vi "LabVIEW.Main.Main_Program.vi"() -> ()   [LabVIEW 2019]
uses:
  LabVIEW.Type Definitions/LabVIEW.Main.Main_Program_Command.ctl
  LabVIEW.Type Definitions/LabVIEW.HTTPs_Client.Command.ctl
  <vilib>/JDP Science/JSONtext/JSONtext.lvlib
panel:
  out "User":T1(array[cluster])
  in  "Test User":bool
  out "Vorgang/Fertigmeldung":T1(array[cluster])
  in  "Test Vorgang/Fertigmeldung":bool
  out "Product/Serial Number":T1(array[cluster])
  in  "Test Product/Serial Number":bool
  out "Label":T1(array[cluster])
  in  "Test Label":bool
  in  "Test Authentication":bool
  out "Authentication":T1(array[cluster])
  out "Größe(n)":i32[](array[numeric])
  out "Table":string[][](table)
  in  "stop":bool caption="Stopp"
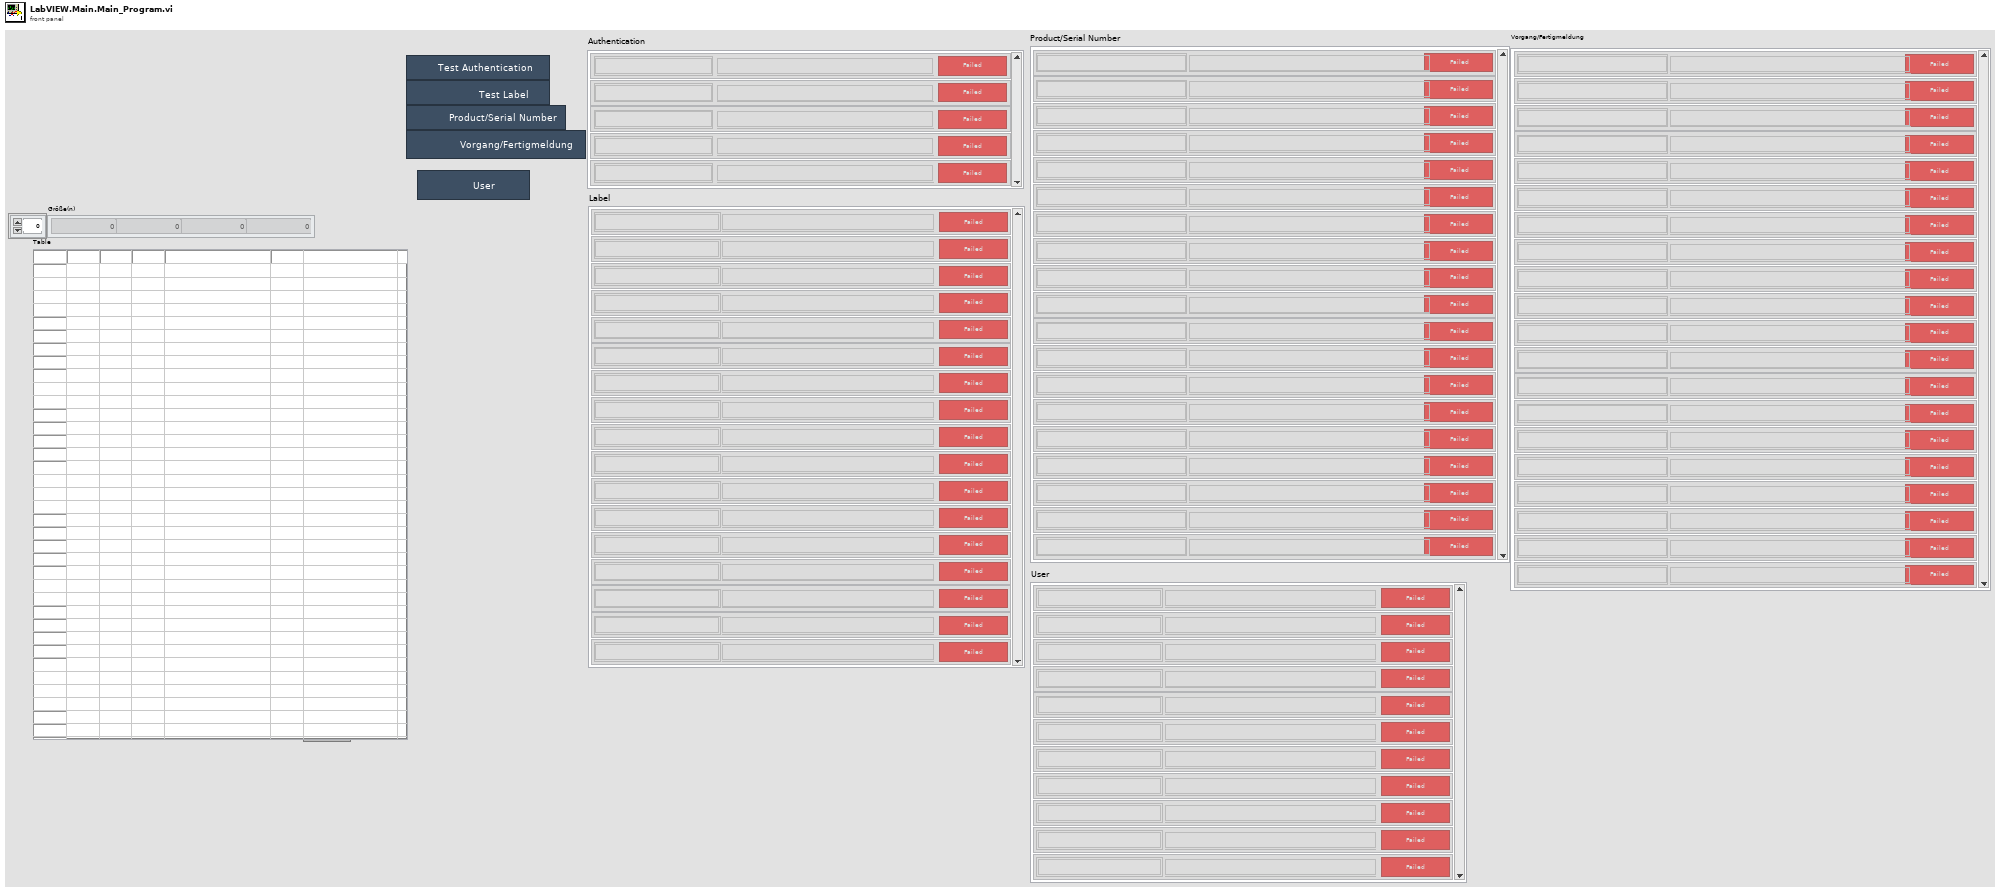
[diagram p1: front panel]
types:
  T1 = cluster{"API Name":string, "API":string, "LED":bool}[]
  T2 = typedef "LabVIEW.Main.Main_Program_Command.ctl" = enum16{"Test Authentication", "Test Label", "Test Product/Serial Number", "Test Vorgang/Fertigmeldung", "Test User"}
  T3 = typedef "LabVIEW.HTTPs_Client.Command.ctl" = enum16{"Initialize HTTPS", "Authentication: Creat a token", "Authentication: Get all tokens", "Authentication: Revoke the token", "Label: Creat a label configuration", "Label: Get all configured labels", "Label: Update the label configuration", "Label: Delete the label configuration", "Label: Creat a colour ribbon", "Label: Update the colour ribbon", "Label: Get all colour ribbons", "Label: Delete the colour ribbon", "Label: Creat a label tape", "Label: Update the label tape", "Label: Get all label tapes", "Label: Delete the label tape", "Label: Get all label parameters", "Product: Get all product informations", "Product: Get all reading steps", "Seriennummer: Update the info text", "Seriennummer: Set all step states open", "Seriennummer: Update step states", "Seriennummer: Get data and steps", "Seriennummer: Get all label configurations", "Seriennummer: Create a text report(Prüfbericht)", "Seriennummer: Get the text report(Prüfbericht)", "Seriennummer: Delete the text report(Prüfbericht)", "Seriennummer: Upload a document(txt file)", "Seriennummer: Get the document", "Seriennummer: Get the document thumbnail", "Seriennummer: Delete the document", "Seriennummer: Bulk lookup", "Vorgang: Update the description text", "Vorgang: Migrate serial numbers to a Vorgang", "Vorgang: Migrate serial numbers to a product revision", "Vorgang: Update step states", "Vorgang: Create test reports(Prüfprotokoll)", "Vorgang: Get basic data", "Vorgang: Get serial number data and steps", "Vorgang: Get all serial numbers", "Vorgang: Generate a CSV file", "Vorgang: Generate an XLSX file", "Vorgang: Get a CSV file(Fertigmeldung report)", "Fertigmeldung: Create a Fertigmeldung", "Fertigmeldung: Revert the Fertigmeldung", "User: Get all users", "User: Update an user", "User: Get a single user", "User: Get all user roles", "User: Update a user role", "User: Get a single user role", "User: Get all permissions", "Search: Get Vorgang/Produkt combinations", "Search: Get Vorgang/Produkt/SN combinations", "Search: Get Seriennummern by Vorgang and Produkt", "Search: Lookup Vorgang", "MAC addresses: Get all reserved MAC addresses", "MAC addresses: Get the most recently reserved MAC addresses", "MAC addresses: Get data for a MAC address", "MAC addresses: Reserve MAC addresses for a Seriennummer", "MAC addresses: Mark a reserved MAC address as flashed", "Deinitialize HTTPs"}
  T4 = enum16{"read csv", "clear csv", "read xlsx", "clear xlsx"}
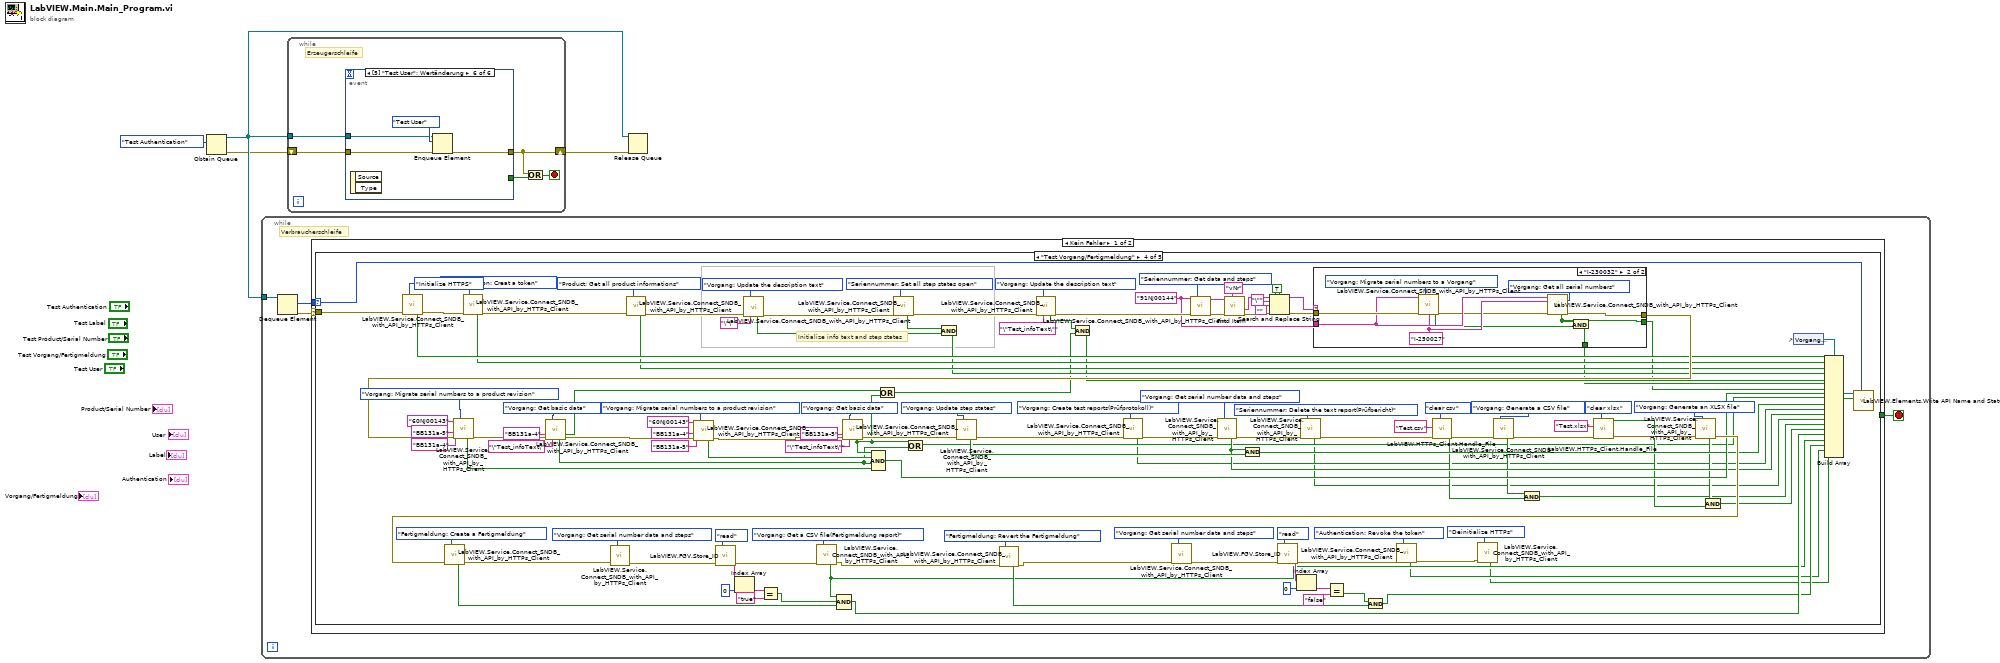
[diagram p0: block diagram]
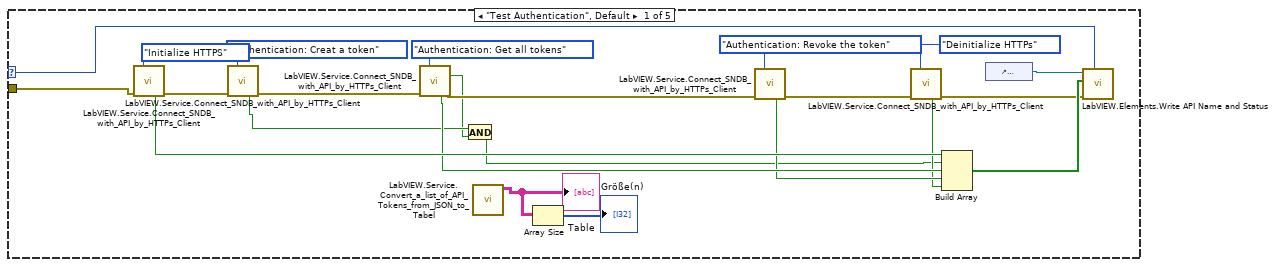
[diagram p2: hidden frame]
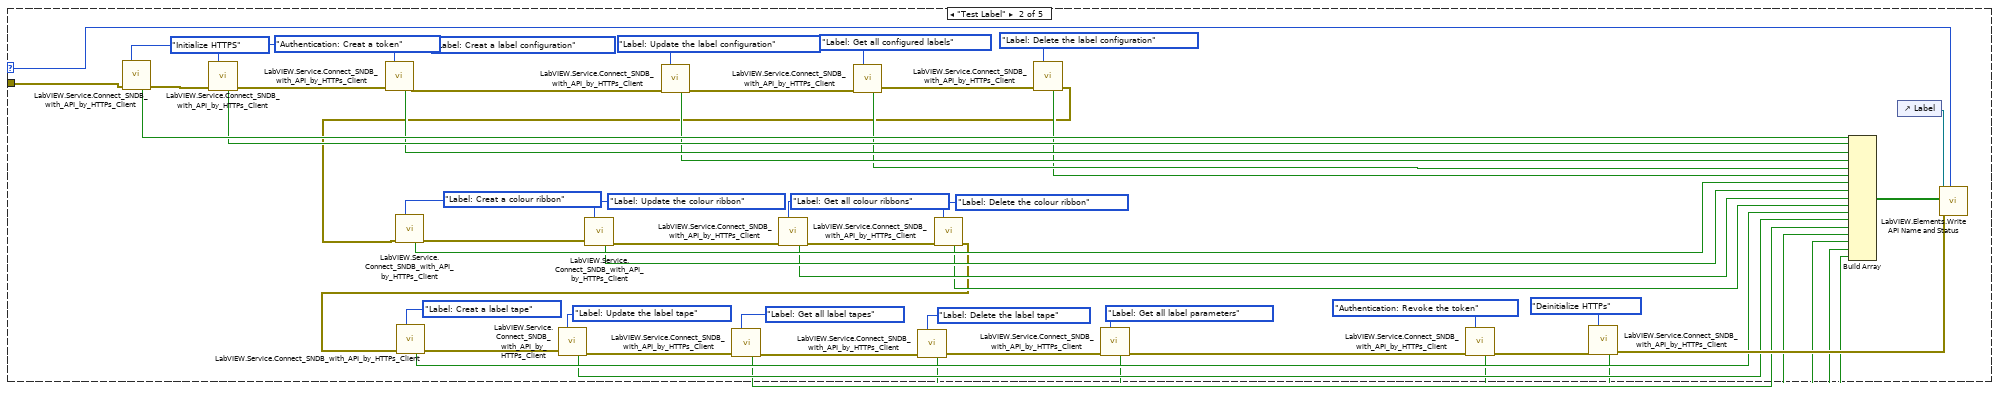
[diagram p3: hidden frame]
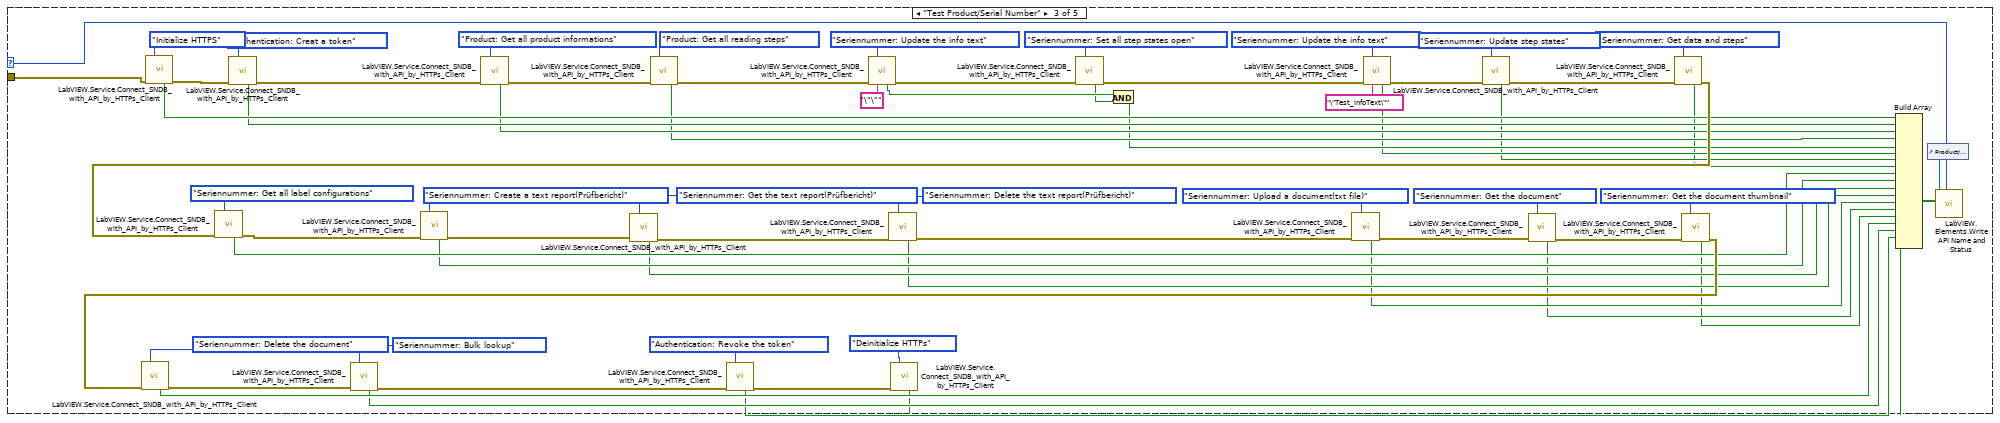
[diagram p4: hidden frame]
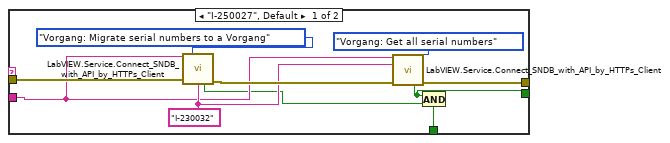
[diagram p5: hidden frame]
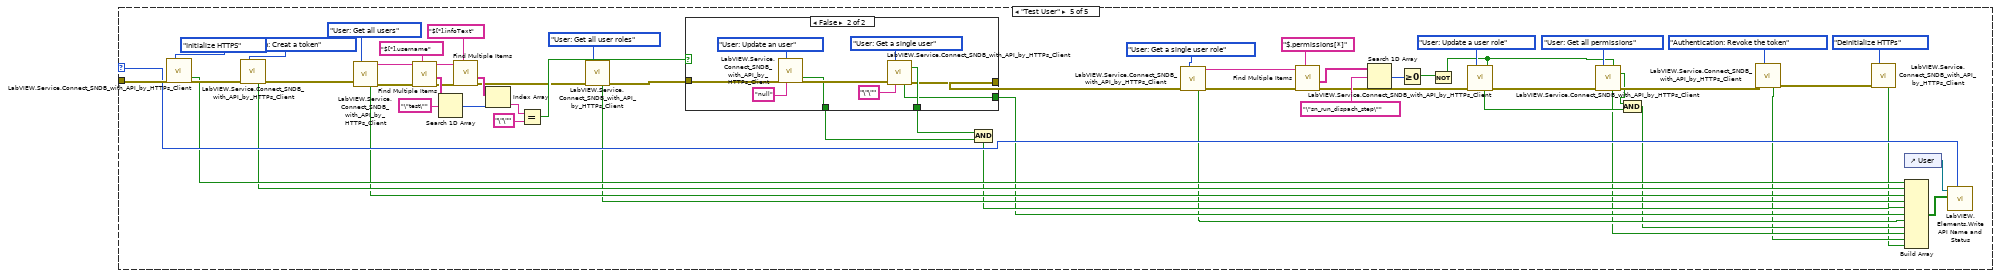
[diagram p6: hidden frame]
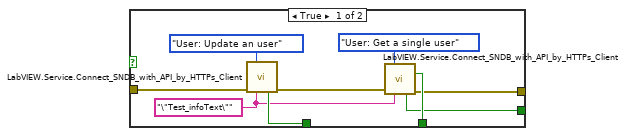
[diagram p7: hidden frame]
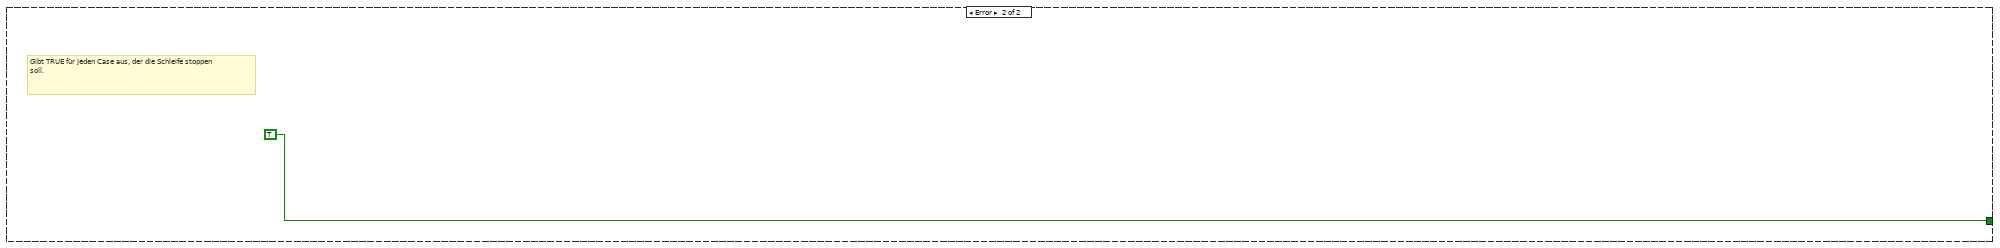
[diagram p8: hidden frame]
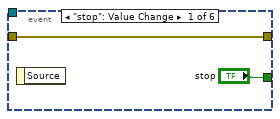
[diagram p9: hidden frame]
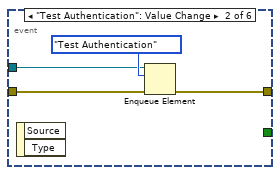
[diagram p10: hidden frame]
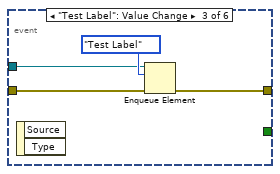
[diagram p11: hidden frame]
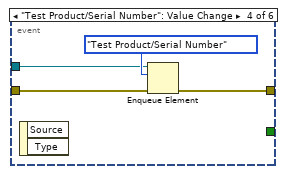
[diagram p12: hidden frame]
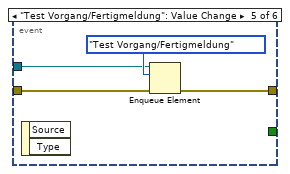
[diagram p13: hidden frame]
diagram:
  n1 = Obtain Queue(element data type=LabVIEW.Main.Main_Program_Command."Test Authentication" ("Command")) -> (queue out=w2:refnum<queue>, error out=w1:errorcluster)  [unwired: 4 in, 1 out]
  n2 = while {
    tunnel: w2 -> [w8]
    stop <- w5 stop-if-true
    # "Verbraucherschleife"
    n3 = Dequeue Element(queue=w8) -> (element=w6:T2, error out=w7:errorcluster)  [unwired: 2 in, 2 out]
    n4 = case shown="Kein Fehler" w7 {
      selector: w7 -> [w9 _]
      tunnel: w6 -> [w10 _]
      tunnel: [_ TRUE] -> w5
      frame No Error {
        n5 = case shown="\"Test Vorgang/Fertigmeldung\"" w10 {
          selector: w10 -> [w14 w34 w112 w199 w333]
          tunnel: w9 -> [w33 w88 w151 w280 w357]
          frame "Test Authentication", Default {
            n6 = call "LabVIEW.Service.Connect_SNDB_with_API_by_HTTPs_Client.vi"("Command"=LabVIEW.HTTPs_Client.Command."Initialize HTTPS", "error in (no error)"=w33) -> ("Successful?"=w26:bool, "error out"=w32:errorcluster)  [unwired: 7 in, 5 out]
            n7 = call "LabVIEW.Service.Connect_SNDB_with_API_by_HTTPs_Client.vi"("Command"=LabVIEW.HTTPs_Client.Command."Authentication: Creat a token", "error in (no error)"=w32) -> ("Successful?"=w13:bool, "error out"=w29:errorcluster)  [unwired: 7 in, 5 out]
            n8 = call "LabVIEW.Service.Connect_SNDB_with_API_by_HTTPs_Client.vi"("Command"=LabVIEW.HTTPs_Client.Command."Authentication: Get all tokens", "error in (no error)"=w29) -> ("Test other steps"=w12:bool, "Successful?"=w25:bool, "error out"=w28:errorcluster)  [unwired: 7 in, 4 out]
            n9 = And(x=w13, y=w12) -> (x .and. y?=w11:bool)
            n10 = call "LabVIEW.Service.Convert_a_list_of_API_Tokens_from_JSON_to_Tabel.vi"() -> ("API Tokens"=w31:string[][])  [unwired: 10 in, 1 out]
            "Table" <- w31
            n11 = Array Size(array=w31) -> (size(s)=→"Größe(n)":i32[])
            n12 = call "LabVIEW.Service.Connect_SNDB_with_API_by_HTTPs_Client.vi"("Command"=LabVIEW.HTTPs_Client.Command."Authentication: Revoke the token", "error in (no error)"=w28) -> ("Successful?"=w24:bool, "error out"=w22:errorcluster)  [unwired: 7 in, 5 out]
            n13 = call "LabVIEW.Service.Connect_SNDB_with_API_by_HTTPs_Client.vi"("Command"=LabVIEW.HTTPs_Client.Command."Deinitialize HTTPs", "error in (no error)"=w22) -> ("Successful?"=w21:bool, "error out"=w20:errorcluster)  [unwired: 7 in, 5 out]
            n14 = Build Array(w26, w11, w25, w24, w21) -> (w23:bool[])
            n15 = control-ref of="Authentication"() -> (w27:refnum<vi>)
            n16 = call "LabVIEW.Elements.Write API Name and Status.vi"("Command"=w14, "Fehler (Eingang, kein Fehler)"=w20, "Status[]"=w23, "Array Reference"=w27) -> ()  [unwired: 7 in, 1 out]
          }
          frame "Test Label" {
            n17 = call "LabVIEW.Service.Connect_SNDB_with_API_by_HTTPs_Client.vi"("Command"=LabVIEW.HTTPs_Client.Command."Initialize HTTPS", "error in (no error)"=w88) -> ("Successful?"=w84:bool, "error out"=w87:errorcluster)  [unwired: 7 in, 5 out]
            n18 = call "LabVIEW.Service.Connect_SNDB_with_API_by_HTTPs_Client.vi"("Command"=LabVIEW.HTTPs_Client.Command."Authentication: Creat a token", "error in (no error)"=w87) -> ("Successful?"=w83:bool, "error out"=w86:errorcluster)  [unwired: 7 in, 5 out]
            n19 = call "LabVIEW.Service.Connect_SNDB_with_API_by_HTTPs_Client.vi"("Command"=LabVIEW.HTTPs_Client.Command."Label: Creat a label configuration", "error in (no error)"=w86) -> ("Successful?"=w82:bool, "error out"=w85:errorcluster)  [unwired: 7 in, 5 out]
            n20 = call "LabVIEW.Service.Connect_SNDB_with_API_by_HTTPs_Client.vi"("Command"=LabVIEW.HTTPs_Client.Command."Label: Update the label configuration", "error in (no error)"=w85) -> ("Successful?"=w81:bool, "error out"=w79:errorcluster)  [unwired: 7 in, 5 out]
            n21 = call "LabVIEW.Service.Connect_SNDB_with_API_by_HTTPs_Client.vi"("Command"=LabVIEW.HTTPs_Client.Command."Label: Get all configured labels", "error in (no error)"=w79) -> ("Successful?"=w78:bool, "error out"=w73:errorcluster)  [unwired: 7 in, 5 out]
            n22 = call "LabVIEW.Service.Connect_SNDB_with_API_by_HTTPs_Client.vi"("Command"=LabVIEW.HTTPs_Client.Command."Label: Delete the label configuration", "error in (no error)"=w73) -> ("Successful?"=w67:bool, "error out"=w60:errorcluster)  [unwired: 7 in, 5 out]
            n23 = call "LabVIEW.Service.Connect_SNDB_with_API_by_HTTPs_Client.vi"("Command"=LabVIEW.HTTPs_Client.Command."Label: Creat a colour ribbon", "error in (no error)"=w60) -> ("Successful?"=w56:bool, "error out"=w59:errorcluster)  [unwired: 7 in, 5 out]
            n24 = call "LabVIEW.Service.Connect_SNDB_with_API_by_HTTPs_Client.vi"("Command"=LabVIEW.HTTPs_Client.Command."Label: Update the colour ribbon", "error in (no error)"=w59) -> ("Successful?"=w55:bool, "error out"=w58:errorcluster)  [unwired: 7 in, 5 out]
            n25 = call "LabVIEW.Service.Connect_SNDB_with_API_by_HTTPs_Client.vi"("Command"=LabVIEW.HTTPs_Client.Command."Label: Get all colour ribbons", "error in (no error)"=w58) -> ("Successful?"=w54:bool, "error out"=w57:errorcluster)  [unwired: 7 in, 5 out]
            n26 = call "LabVIEW.Service.Connect_SNDB_with_API_by_HTTPs_Client.vi"("Command"=LabVIEW.HTTPs_Client.Command."Label: Delete the colour ribbon", "error in (no error)"=w57) -> ("Successful?"=w53:bool, "error out"=w45:errorcluster)  [unwired: 7 in, 5 out]
            n27 = call "LabVIEW.Service.Connect_SNDB_with_API_by_HTTPs_Client.vi"("Command"=LabVIEW.HTTPs_Client.Command."Label: Creat a label tape", "error in (no error)"=w45) -> ("Successful?"=w44:bool, "error out"=w48:errorcluster)  [unwired: 7 in, 5 out]
            n28 = call "LabVIEW.Service.Connect_SNDB_with_API_by_HTTPs_Client.vi"("Command"=LabVIEW.HTTPs_Client.Command."Label: Update the label tape", "error in (no error)"=w48) -> ("Successful?"=w43:bool, "error out"=w47:errorcluster)  [unwired: 7 in, 5 out]
            n29 = call "LabVIEW.Service.Connect_SNDB_with_API_by_HTTPs_Client.vi"("Command"=LabVIEW.HTTPs_Client.Command."Label: Get all label tapes", "error in (no error)"=w47) -> ("Successful?"=w42:bool, "error out"=w46:errorcluster)  [unwired: 7 in, 5 out]
            n30 = call "LabVIEW.Service.Connect_SNDB_with_API_by_HTTPs_Client.vi"("Command"=LabVIEW.HTTPs_Client.Command."Label: Delete the label tape", "error in (no error)"=w46) -> ("Successful?"=w41:bool, "error out"=w40:errorcluster)  [unwired: 7 in, 5 out]
            n31 = call "LabVIEW.Service.Connect_SNDB_with_API_by_HTTPs_Client.vi"("Command"=LabVIEW.HTTPs_Client.Command."Label: Get all label parameters", "error in (no error)"=w40) -> ("Successful?"=w37:bool, "error out"=w39:errorcluster)  [unwired: 7 in, 5 out]
            n32 = call "LabVIEW.Service.Connect_SNDB_with_API_by_HTTPs_Client.vi"("Command"=LabVIEW.HTTPs_Client.Command."Authentication: Revoke the token", "error in (no error)"=w39) -> ("Successful?"=w36:bool, "error out"=w70:errorcluster)  [unwired: 7 in, 5 out]
            n33 = call "LabVIEW.Service.Connect_SNDB_with_API_by_HTTPs_Client.vi"("Command"=LabVIEW.HTTPs_Client.Command."Deinitialize HTTPs", "error in (no error)"=w70) -> ("Successful?"=w35:bool, "error out"=w68:errorcluster)  [unwired: 7 in, 5 out]
            n34 = Build Array(w84, w83, w82, w81, w78, w67, w56, w55, w54, w53, w44, w43, w42, w41, w37, w36, w35) -> (w80:bool[])
            n35 = control-ref of="Label"() -> (w69:refnum<vi>)
            n36 = call "LabVIEW.Elements.Write API Name and Status.vi"("Command"=w34, "Fehler (Eingang, kein Fehler)"=w68, "Status[]"=w80, "Array Reference"=w69) -> ()  [unwired: 7 in, 1 out]
          }
          frame "Test Product/Serial Number" {
            n37 = call "LabVIEW.Service.Connect_SNDB_with_API_by_HTTPs_Client.vi"("Command"=LabVIEW.HTTPs_Client.Command."Initialize HTTPS", "error in (no error)"=w151) -> ("Successful?"=w110:bool, "error out"=w154:errorcluster)  [unwired: 7 in, 5 out]
            n38 = call "LabVIEW.Service.Connect_SNDB_with_API_by_HTTPs_Client.vi"("Command"=LabVIEW.HTTPs_Client.Command."Authentication: Creat a token", "error in (no error)"=w154) -> ("Successful?"=w109:bool, "error out"=w148:errorcluster)  [unwired: 7 in, 5 out]
            n39 = call "LabVIEW.Service.Connect_SNDB_with_API_by_HTTPs_Client.vi"("Command"=LabVIEW.HTTPs_Client.Command."Product: Get all product informations", "error in (no error)"=w148) -> ("Successful?"=w108:bool, "error out"=w147:errorcluster)  [unwired: 7 in, 5 out]
            n40 = call "LabVIEW.Service.Connect_SNDB_with_API_by_HTTPs_Client.vi"("Command"=LabVIEW.HTTPs_Client.Command."Product: Get all reading steps", "error in (no error)"=w147) -> ("Successful?"=w107:bool, "error out"=w144:errorcluster)  [unwired: 7 in, 5 out]
            n41 = call "LabVIEW.Service.Connect_SNDB_with_API_by_HTTPs_Client.vi"("Command"=LabVIEW.HTTPs_Client.Command."Seriennummer: Update the info text", "error in (no error)"=w144, "Info text"="\"\"" ("SN: Info text")) -> ("Successful?"=w106:bool, "error out"=w142:errorcluster)  [unwired: 6 in, 5 out]
            n42 = call "LabVIEW.Service.Connect_SNDB_with_API_by_HTTPs_Client.vi"("Command"=LabVIEW.HTTPs_Client.Command."Seriennummer: Set all step states open", "error in (no error)"=w142) -> ("Successful?"=w105:bool, "error out"=w140:errorcluster)  [unwired: 7 in, 5 out]
            n43 = And(x=w106, y=w105) -> (x .and. y?=w104:bool)
            n44 = call "LabVIEW.Service.Connect_SNDB_with_API_by_HTTPs_Client.vi"("Command"=LabVIEW.HTTPs_Client.Command."Seriennummer: Update the info text", "error in (no error)"=w140, "Info text"="\"Test_infoText\"" ("SN: Info text")) -> ("Successful?"=w103:bool, "error out"=w138:errorcluster)  [unwired: 6 in, 5 out]
            n45 = call "LabVIEW.Service.Connect_SNDB_with_API_by_HTTPs_Client.vi"("Command"=LabVIEW.HTTPs_Client.Command."Seriennummer: Update step states", "error in (no error)"=w138) -> ("Successful?"=w102:bool, "error out"=w136:errorcluster)  [unwired: 7 in, 5 out]
            n46 = call "LabVIEW.Service.Connect_SNDB_with_API_by_HTTPs_Client.vi"("Command"=LabVIEW.HTTPs_Client.Command."Seriennummer: Get data and steps", "error in (no error)"=w136) -> ("Successful?"=w101:bool, "error out"=w115:errorcluster)  [unwired: 7 in, 5 out]
            n47 = call "LabVIEW.Service.Connect_SNDB_with_API_by_HTTPs_Client.vi"("Command"=LabVIEW.HTTPs_Client.Command."Seriennummer: Get all label configurations", "error in (no error)"=w115) -> ("Successful?"=w100:bool, "error out"=w132:errorcluster)  [unwired: 7 in, 5 out]
            n48 = call "LabVIEW.Service.Connect_SNDB_with_API_by_HTTPs_Client.vi"("Command"=LabVIEW.HTTPs_Client.Command."Seriennummer: Create a text report(Prüfbericht)", "error in (no error)"=w132) -> ("Successful?"=w99:bool, "error out"=w131:errorcluster)  [unwired: 7 in, 5 out]
            n49 = call "LabVIEW.Service.Connect_SNDB_with_API_by_HTTPs_Client.vi"("Command"=LabVIEW.HTTPs_Client.Command."Seriennummer: Get the text report(Prüfbericht)", "error in (no error)"=w131) -> ("Successful?"=w98:bool, "error out"=w129:errorcluster)  [unwired: 7 in, 5 out]
            n50 = call "LabVIEW.Service.Connect_SNDB_with_API_by_HTTPs_Client.vi"("Command"=LabVIEW.HTTPs_Client.Command."Seriennummer: Delete the text report(Prüfbericht)", "error in (no error)"=w129) -> ("Successful?"=w97:bool, "error out"=w128:errorcluster)  [unwired: 7 in, 5 out]
            n51 = call "LabVIEW.Service.Connect_SNDB_with_API_by_HTTPs_Client.vi"("Command"=LabVIEW.HTTPs_Client.Command."Seriennummer: Upload a document(txt file)", "error in (no error)"=w128) -> ("Successful?"=w96:bool, "error out"=w126:errorcluster)  [unwired: 7 in, 5 out]
            n52 = call "LabVIEW.Service.Connect_SNDB_with_API_by_HTTPs_Client.vi"("Command"=LabVIEW.HTTPs_Client.Command."Seriennummer: Get the document", "error in (no error)"=w126) -> ("Successful?"=w95:bool, "error out"=w123:errorcluster)  [unwired: 7 in, 5 out]
            n53 = call "LabVIEW.Service.Connect_SNDB_with_API_by_HTTPs_Client.vi"("Command"=LabVIEW.HTTPs_Client.Command."Seriennummer: Get the document thumbnail", "error in (no error)"=w123) -> ("Successful?"=w94:bool, "error out"=w114:errorcluster)  [unwired: 7 in, 5 out]
            n54 = call "LabVIEW.Service.Connect_SNDB_with_API_by_HTTPs_Client.vi"("Command"=LabVIEW.HTTPs_Client.Command."Seriennummer: Delete the document", "error in (no error)"=w114) -> ("Successful?"=w93:bool, "error out"=w118:errorcluster)  [unwired: 7 in, 5 out]
            n55 = call "LabVIEW.Service.Connect_SNDB_with_API_by_HTTPs_Client.vi"("Command"=LabVIEW.HTTPs_Client.Command."Seriennummer: Bulk lookup", "error in (no error)"=w118) -> ("Successful?"=w92:bool, "error out"=w117:errorcluster)  [unwired: 7 in, 5 out]
            n56 = call "LabVIEW.Service.Connect_SNDB_with_API_by_HTTPs_Client.vi"("Command"=LabVIEW.HTTPs_Client.Command."Authentication: Revoke the token", "error in (no error)"=w117) -> ("Successful?"=w91:bool, "error out"=w116:errorcluster)  [unwired: 7 in, 5 out]
            n57 = call "LabVIEW.Service.Connect_SNDB_with_API_by_HTTPs_Client.vi"("Command"=LabVIEW.HTTPs_Client.Command."Deinitialize HTTPs", "error in (no error)"=w116) -> ("Successful?"=w90:bool)  [unwired: 7 in, 6 out]
            n58 = Build Array(w110, w109, w108, w107, w104, w103, w102, w101, w100, w99, w98, w97, w96, w95, w94, w93, w92, w91, w90) -> (w113:bool[])
            n59 = control-ref of="Product/Serial Number"() -> (w111:refnum<vi>)
            n60 = call "LabVIEW.Elements.Write API Name and Status.vi"("Command"=w112, "Status[]"=w113, "Array Reference"=w111) -> ()  [unwired: 8 in, 1 out]
          }
          frame "Test Vorgang/Fertigmeldung" {
            w267 = TRUE ("Alle ersetzen? (F)")
            w261 = "91NJ00144" ("SN")
            # "Initialize info text and step states"
            n61 = call "LabVIEW.Service.Connect_SNDB_with_API_by_HTTPs_Client.vi"("Command"=LabVIEW.HTTPs_Client.Command."Initialize HTTPS", "error in (no error)"=w280) -> ("Successful?"=w197:bool, "error out"=w283:errorcluster)  [unwired: 7 in, 5 out]
            n62 = call "LabVIEW.Service.Connect_SNDB_with_API_by_HTTPs_Client.vi"("Command"=LabVIEW.HTTPs_Client.Command."Authentication: Creat a token", "error in (no error)"=w283) -> ("Successful?"=w196:bool, "error out"=w249:errorcluster)  [unwired: 7 in, 5 out]
            n63 = call "LabVIEW.Service.Connect_SNDB_with_API_by_HTTPs_Client.vi"("Command"=LabVIEW.HTTPs_Client.Command."Product: Get all product informations", "error in (no error)"=w249) -> ("Successful?"=w195:bool, "error out"=w248:errorcluster)  [unwired: 7 in, 5 out]
            n64 = call "LabVIEW.Service.Connect_SNDB_with_API_by_HTTPs_Client.vi"("Command"=LabVIEW.HTTPs_Client.Command."Vorgang: Update the description text", "error in (no error)"=w248, "Info text"="\"\"") -> ("Successful?"=w194:bool, "error out"=w276:errorcluster)  [unwired: 6 in, 5 out]
            n65 = call "LabVIEW.Service.Connect_SNDB_with_API_by_HTTPs_Client.vi"("Command"=LabVIEW.HTTPs_Client.Command."Seriennummer: Set all step states open", "error in (no error)"=w276) -> ("Successful?"=w193:bool, "error out"=w273:errorcluster)  [unwired: 7 in, 5 out]
            n66 = And(x=w193, y=w194) -> (x .and. y?=w192:bool)
            n67 = call "LabVIEW.Service.Connect_SNDB_with_API_by_HTTPs_Client.vi"("Command"=LabVIEW.HTTPs_Client.Command."Vorgang: Update the description text", "error in (no error)"=w273, "Info text"="\"Test_infoText\"") -> ("Successful?"=w190:bool, "error out"=w271:errorcluster)  [unwired: 6 in, 5 out]
            n68 = call "LabVIEW.Service.Connect_SNDB_with_API_by_HTTPs_Client.vi"("SN"=w261, "Command"=LabVIEW.HTTPs_Client.Command."Seriennummer: Get data and steps", "error in (no error)"=w271) -> ("Body"=w269:string, "error out"=w270:errorcluster)  [unwired: 6 in, 5 out]
            n69 = call <vilib>:"Find Item.vi"("$Path or Item Name"="vNr", "error in (no error)"=w270, "JSON"=w269) -> ("error out"=w263:errorcluster, "<JSON>"=w264:string)  [unwired: 5 in, 2 out]
            n70 = Search and Replace String(replace all?=w267, case sensitive?=w267, input string=w264, search string="\"" ("Such-String"), replace string="", error in=w263) -> (result string=w262:string, error out=w260:errorcluster)  [unwired: 2 in, 2 out]
            n71 = case shown="\"I-230032\"" w262 {
              tunnel: w261 -> [w287 w299]
              tunnel: w260 -> [w293 w302]
              tunnel: [w289 w300] -> w255
              tunnel: [w285 w295] -> w188
              tunnel: [w284 w294] -> w187
              frame "I-250027", Default {
                w288 = "I-230032" ("Migrated Vorgang")
                n72 = call "LabVIEW.Service.Connect_SNDB_with_API_by_HTTPs_Client.vi"("SN"=w287, "Command"=LabVIEW.HTTPs_Client.Command."Vorgang: Migrate serial numbers to a Vorgang", "error in (no error)"=w293, "Migrated Vorgang"=w288) -> ("Successful?"=w286:bool, "error out"=w290:errorcluster)  [unwired: 5 in, 5 out]
                n73 = call "LabVIEW.Service.Connect_SNDB_with_API_by_HTTPs_Client.vi"("SN"=w287, "Command"=LabVIEW.HTTPs_Client.Command."Vorgang: Get all serial numbers", "VrN"=w288, "error in (no error)"=w290) -> ("Successful?"=w284:bool, "error out"=w289:errorcluster)  [unwired: 5 in, 5 out]
                n74 = And(x=w284, y=w286) -> (x .and. y?=w285:bool)
              }
              frame "I-230032" {
                w298 = "I-250027" ("Migrated Vorgang")
                n75 = call "LabVIEW.Service.Connect_SNDB_with_API_by_HTTPs_Client.vi"("SN"=w299, "Command"=LabVIEW.HTTPs_Client.Command."Vorgang: Migrate serial numbers to a Vorgang", "error in (no error)"=w302, "Migrated Vorgang"=w298) -> ("Successful?"=w296:bool, "error out"=w297:errorcluster)  [unwired: 5 in, 5 out]
                n76 = call "LabVIEW.Service.Connect_SNDB_with_API_by_HTTPs_Client.vi"("SN"=w299, "Command"=LabVIEW.HTTPs_Client.Command."Vorgang: Get all serial numbers", "VrN"=w298, "error in (no error)"=w297) -> ("Successful?"=w294:bool, "error out"=w300:errorcluster)  [unwired: 5 in, 5 out]
                n77 = And(x=w294, y=w296) -> (x .and. y?=w295:bool)
              }
            }
            n78 = call "LabVIEW.Service.Connect_SNDB_with_API_by_HTTPs_Client.vi"("SN"="60NJ00143", "Command"=LabVIEW.HTTPs_Client.Command."Vorgang: Migrate serial numbers to a product revision", "Old Product"="BB131a-5", "Changed Product"="BB131a-4", "error in (no error)"=w255) -> ("Successful?"=w184:bool, "error out"=w253:errorcluster)  [unwired: 4 in, 5 out]
            n79 = call "LabVIEW.Service.Connect_SNDB_with_API_by_HTTPs_Client.vi"("Command"=LabVIEW.HTTPs_Client.Command."Vorgang: Get basic data", "Changed Product"="BB131a-4", "error in (no error)"=w253, "Info text"="\"Test_infoText\"") -> ("Successful?"=w169:bool, "error out"=w242:errorcluster)  [unwired: 5 in, 5 out]
            n80 = call "LabVIEW.Service.Connect_SNDB_with_API_by_HTTPs_Client.vi"("SN"="60NJ00143", "Command"=LabVIEW.HTTPs_Client.Command."Vorgang: Migrate serial numbers to a product revision", "Old Product"="BB131a-4", "Changed Product"="BB131a-5", "error in (no error)"=w242) -> ("Successful?"=w185:bool, "error out"=w238:errorcluster)  [unwired: 4 in, 5 out]
            n81 = call "LabVIEW.Service.Connect_SNDB_with_API_by_HTTPs_Client.vi"("Command"=LabVIEW.HTTPs_Client.Command."Vorgang: Get basic data", "Changed Product"="BB131a-5", "error in (no error)"=w238, "Info text"="\"Test_infoText\"") -> ("Successful?"=w170:bool, "error out"=w186:errorcluster)  [unwired: 5 in, 5 out]
            n82 = Compound Arithmetic op=AND ("Mehrfacharithmetik")(w170, w185, w169, w184) -> (w183:bool)
            n83 = Or(x=w169, y=w170) -> (x .or. y?=w191:bool)
            n84 = Or(x=w170, y=w169) -> (x .or. y?=w168:bool)
            n85 = call "LabVIEW.Service.Connect_SNDB_with_API_by_HTTPs_Client.vi"("Command"=LabVIEW.HTTPs_Client.Command."Vorgang: Update step states", "error in (no error)"=w186) -> ("Successful?"=w182:bool, "error out"=w236:errorcluster)  [unwired: 7 in, 5 out]
            n86 = And(x=w190, y=w191) -> (x .and. y?=w189:bool)
            n87 = call "LabVIEW.Service.Connect_SNDB_with_API_by_HTTPs_Client.vi"("Command"=LabVIEW.HTTPs_Client.Command."Vorgang: Create test reports(Prüfprotokoll)", "error in (no error)"=w236) -> ("Successful?"=w167:bool, "error out"=w235:errorcluster)  [unwired: 7 in, 5 out]
            n88 = call "LabVIEW.Service.Connect_SNDB_with_API_by_HTTPs_Client.vi"("Command"=LabVIEW.HTTPs_Client.Command."Vorgang: Get serial number data and steps", "error in (no error)"=w235) -> ("Successful?"=w180:bool, "error out"=w165:errorcluster)  [unwired: 7 in, 5 out]
            n89 = And(x=w180, y=w182) -> (x .and. y?=w181:bool)
            n90 = call "LabVIEW.Service.Connect_SNDB_with_API_by_HTTPs_Client.vi"("Command"=LabVIEW.HTTPs_Client.Command."Seriennummer: Delete the text report(Prüfbericht)", "error in (no error)"=w165) -> ("Successful?"=w162:bool, "error out"=w164:errorcluster)  [unwired: 7 in, 5 out]
            n91 = call "LabVIEW.HTTPs_Client.Handle_File.vi"("Command"=T4."clear csv", "Fehler (Eingang, kein Fehler)"=w164, "File name"="Test.csv") -> ("Fehler (Ausgang)"=w232:errorcluster, "Successful?"=w178:bool)  [unwired: 7 in]
            n92 = call "LabVIEW.Service.Connect_SNDB_with_API_by_HTTPs_Client.vi"("Command"=LabVIEW.HTTPs_Client.Command."Vorgang: Generate a CSV file", "error in (no error)"=w232) -> ("Successful?"=w179:bool, "error out"=w230:errorcluster)  [unwired: 7 in, 5 out]
            n93 = And(x=w179, y=w178) -> (x .and. y?=w160:bool)
            n94 = call "LabVIEW.HTTPs_Client.Handle_File.vi"("Command"=T4."clear xlsx", "Fehler (Eingang, kein Fehler)"=w230, "File name"="Test.xlsx") -> ("Fehler (Ausgang)"=w227:errorcluster, "Successful?"=w176:bool)  [unwired: 7 in]
            n95 = call "LabVIEW.Service.Connect_SNDB_with_API_by_HTTPs_Client.vi"("Command"=LabVIEW.HTTPs_Client.Command."Vorgang: Generate an XLSX file", "error in (no error)"=w227) -> ("Successful?"=w177:bool, "error out"=w223:errorcluster)  [unwired: 7 in, 5 out]
            n96 = call "LabVIEW.Service.Connect_SNDB_with_API_by_HTTPs_Client.vi"("Command"=LabVIEW.HTTPs_Client.Command."Fertigmeldung: Create a Fertigmeldung", "error in (no error)"=w223) -> ("Successful?"=w174:bool, "error out"=w222:errorcluster)  [unwired: 7 in, 5 out]
            n97 = call "LabVIEW.Service.Connect_SNDB_with_API_by_HTTPs_Client.vi"("Command"=LabVIEW.HTTPs_Client.Command."Vorgang: Get serial number data and steps", "error in (no error)"=w222) -> ("error out"=w220:errorcluster)  [unwired: 7 in, 6 out]
            n98 = call "LabVIEW.FGV.Store_ID.vi"("Command"=enum16{"clear", "write", "read"}."read", "error in (no error)"=w220) -> ("Fertigmeldung out[]"=w219:string[], "error out"=w214:errorcluster)  [unwired: 8 in, 4 out]
            n99 = Index Array(array=w219, index=0 ("Index")) -> (element=w217:string)
            n100 = Equal?(x=w217, y="true") -> (x = y?=w175:bool)
            n101 = call "LabVIEW.Service.Connect_SNDB_with_API_by_HTTPs_Client.vi"("Command"=LabVIEW.HTTPs_Client.Command."Vorgang: Get a CSV file(Fertigmeldung report)", "error in (no error)"=w214) -> ("Successful?"=w158:bool, "error out"=w212:errorcluster)  [unwired: 7 in, 5 out]
            n102 = Compound Arithmetic op=AND ("Mehrfacharithmetik")(w158, w175, w174) -> (w159:bool)
            n103 = call "LabVIEW.Service.Connect_SNDB_with_API_by_HTTPs_Client.vi"("Command"=LabVIEW.HTTPs_Client.Command."Fertigmeldung: Revert the Fertigmeldung", "error in (no error)"=w212) -> ("Successful?"=w172:bool, "error out"=w207:errorcluster)  [unwired: 7 in, 5 out]
            n104 = call "LabVIEW.Service.Connect_SNDB_with_API_by_HTTPs_Client.vi"("Command"=LabVIEW.HTTPs_Client.Command."Vorgang: Get serial number data and steps", "error in (no error)"=w207) -> ("error out"=w209:errorcluster)  [unwired: 7 in, 6 out]
            n105 = call "LabVIEW.FGV.Store_ID.vi"("Command"=enum16{"clear", "write", "read"}."read", "error in (no error)"=w209) -> ("Fertigmeldung out[]"=w210:string[], "error out"=w203:errorcluster)  [unwired: 8 in, 4 out]
            n106 = Index Array(array=w210, index=0 ("Index")) -> (element=w206:string)
            n107 = Equal?(x=w206, y="false") -> (x = y?=w173:bool)
            n108 = And(x=w173, y=w172) -> (x .and. y?=w157:bool)
            n109 = call "LabVIEW.Service.Connect_SNDB_with_API_by_HTTPs_Client.vi"("Command"=LabVIEW.HTTPs_Client.Command."Authentication: Revoke the token", "error in (no error)"=w203) -> ("Successful?"=w156:bool, "error out"=w200:errorcluster)  [unwired: 7 in, 5 out]
            n110 = call "LabVIEW.Service.Connect_SNDB_with_API_by_HTTPs_Client.vi"("Command"=LabVIEW.HTTPs_Client.Command."Deinitialize HTTPs", "error in (no error)"=w200) -> ("Successful?"=w155:bool)  [unwired: 7 in, 6 out]
            n111 = And(x=w177, y=w176) -> (x .and. y?=w161:bool)
            n112 = control-ref of="Vorgang/Fertigmeldung"() -> (w198:refnum<vi>)
            n113 = Build Array(w197, w196, w195, w192, w189, w188, w187, w183, w168, w181, w167, w180, w162, w160, w161, w159, w158, w157, w156, w155) -> (w171:bool[])
            n114 = call "LabVIEW.Elements.Write API Name and Status.vi"("Command"=w199, "Status[]"=w171, "Array Reference"=w198) -> ()  [unwired: 8 in, 1 out]
          }
          frame "Test User" {
            n115 = call "LabVIEW.Service.Connect_SNDB_with_API_by_HTTPs_Client.vi"("Command"=LabVIEW.HTTPs_Client.Command."Initialize HTTPS", "error in (no error)"=w357) -> ("Successful?"=w332:bool, "error out"=w360:errorcluster)  [unwired: 7 in, 5 out]
            n116 = call "LabVIEW.Service.Connect_SNDB_with_API_by_HTTPs_Client.vi"("Command"=LabVIEW.HTTPs_Client.Command."Authentication: Creat a token", "error in (no error)"=w360) -> ("Successful?"=w331:bool, "error out"=w355:errorcluster)  [unwired: 7 in, 5 out]
            n117 = call "LabVIEW.Service.Connect_SNDB_with_API_by_HTTPs_Client.vi"("Command"=LabVIEW.HTTPs_Client.Command."User: Get all users", "error in (no error)"=w355) -> ("Body"=w319:string, "Successful?"=w330:bool, "error out"=w321:errorcluster)  [unwired: 7 in, 4 out]
            n118 = call <vilib>:"Find Multiple Items.vi"("$Path or Item Name"="$[*].username", "error in (no error)"=w321, "JSON"=w319) -> ("error out"=w320:errorcluster, "<JSON>"=w323:string[])  [unwired: 5 in, 2 out]
            n119 = Search 1D Array(1D array=w323, element="\"test\"" ("Element")) -> (index of element=w317:i32)  [unwired: 1 in]
            n120 = call <vilib>:"Find Multiple Items.vi"("$Path or Item Name"="$[*].infoText", "error in (no error)"=w320, "JSON"=w319) -> ("error out"=w313:errorcluster, "<JSON>"=w318:string[])  [unwired: 5 in, 2 out]
            n121 = Index Array(array=w318, index=w317) -> (element=w316:string)
            n122 = Equal?(x=w316, y="\"\"" ("Info text")) -> (x = y?=w325:bool)
            n123 = call "LabVIEW.Service.Connect_SNDB_with_API_by_HTTPs_Client.vi"("Command"=LabVIEW.HTTPs_Client.Command."User: Get all user roles", "error in (no error)"=w313) -> ("Successful?"=w311:bool, "error out"=w312:errorcluster)  [unwired: 7 in, 5 out]
            n124 = case shown="False" w325 {
              tunnel: [w366 w376] -> w337
              tunnel: [w365 w375] -> w336
              tunnel: w312 -> [w364 w374]
              tunnel: [w362 w371] -> w315
              tunnel: [w361 w370] -> w309
              frame True {
                w363 = "\"Test_infoText\"" ("Info text")
                n125 = call "LabVIEW.Service.Connect_SNDB_with_API_by_HTTPs_Client.vi"("Command"=LabVIEW.HTTPs_Client.Command."User: Update an user", "error in (no error)"=w364, "Info text"=w363) -> ("Successful?"=w366:bool, "error out"=w367:errorcluster)  [unwired: 6 in, 5 out]
                n126 = call "LabVIEW.Service.Connect_SNDB_with_API_by_HTTPs_Client.vi"("Command"=LabVIEW.HTTPs_Client.Command."User: Get a single user", "error in (no error)"=w367, "Info text"=w363) -> ("Test other steps"=w365:bool, "Successful?"=w361:bool, "error out"=w362:errorcluster)  [unwired: 6 in, 4 out]
              }
              frame False {
                n127 = call "LabVIEW.Service.Connect_SNDB_with_API_by_HTTPs_Client.vi"("Command"=LabVIEW.HTTPs_Client.Command."User: Update an user", "error in (no error)"=w374, "Info text"="null") -> ("Successful?"=w376:bool, "error out"=w377:errorcluster)  [unwired: 6 in, 5 out]
                n128 = call "LabVIEW.Service.Connect_SNDB_with_API_by_HTTPs_Client.vi"("Command"=LabVIEW.HTTPs_Client.Command."User: Get a single user", "error in (no error)"=w377, "Info text"="\"\"") -> ("Test other steps"=w375:bool, "Successful?"=w370:bool, "error out"=w371:errorcluster)  [unwired: 6 in, 4 out]
              }
            }
            n129 = Compound Arithmetic op=AND ("Mehrfacharithmetik")(w336, w337) -> (w310:bool)
            n130 = call "LabVIEW.Service.Connect_SNDB_with_API_by_HTTPs_Client.vi"("Command"=LabVIEW.HTTPs_Client.Command."User: Get a single user role", "error in (no error)"=w315) -> ("Body"=w351:string, "Successful?"=w308:bool, "error out"=w352:errorcluster)  [unwired: 7 in, 4 out]
            n131 = call <vilib>:"Find Multiple Items.vi"("$Path or Item Name"="$.permissions[*]", "error in (no error)"=w352, "JSON"=w351) -> ("error out"=w345:errorcluster, "<JSON>"=w350:string[])  [unwired: 5 in, 2 out]
            n132 = Search 1D Array(1D array=w350, element="\"sn_run_dispach_step\"" ("Neues Element/Teil-Array")) -> (index of element=w348:i32)  [unwired: 1 in]
            n133 = Greater Or Equal To 0?(x=w348) -> (x >= 0?=w346:bool)
            n134 = Not(x=w346) -> (.not. x?=w343:bool)
            n135 = call "LabVIEW.Service.Connect_SNDB_with_API_by_HTTPs_Client.vi"("Command"=LabVIEW.HTTPs_Client.Command."User: Update a user role", "User Update user role\"sn_run_dispach_step\""=w343, "error in (no error)"=w345) -> ("Successful?"=w334:bool, "error out"=w342:errorcluster)  [unwired: 6 in, 5 out]
            n136 = call "LabVIEW.Service.Connect_SNDB_with_API_by_HTTPs_Client.vi"("Command"=LabVIEW.HTTPs_Client.Command."User: Get all permissions", "User Update user role\"sn_run_dispach_step\""=w343, "error in (no error)"=w342) -> ("Test other steps"=w335:bool, "Successful?"=w306:bool, "error out"=w341:errorcluster)  [unwired: 6 in, 4 out]
            n137 = And(x=w335, y=w334) -> (x .and. y?=w307:bool)
            n138 = call "LabVIEW.Service.Connect_SNDB_with_API_by_HTTPs_Client.vi"("Command"=LabVIEW.HTTPs_Client.Command."Authentication: Revoke the token", "error in (no error)"=w341) -> ("Successful?"=w305:bool, "error out"=w339:errorcluster)  [unwired: 7 in, 5 out]
            n139 = call "LabVIEW.Service.Connect_SNDB_with_API_by_HTTPs_Client.vi"("Command"=LabVIEW.HTTPs_Client.Command."Deinitialize HTTPs", "error in (no error)"=w339) -> ("Successful?"=w304:bool)  [unwired: 7 in, 6 out]
            n140 = control-ref of="User"() -> (w328:refnum<vi>)
            n141 = Build Array(w332, w331, w330, w311, w310, w309, w308, w307, w306, w305, w304) -> (w329:bool[])
            n142 = call "LabVIEW.Elements.Write API Name and Status.vi"("Command"=w333, "Status[]"=w329, "Array Reference"=w328) -> ()  [unwired: 8 in, 1 out]
          }
        }
      }
      frame Error {
        # "Gibt TRUE für jeden Case aus, der die Schleife stoppen soll."
      }
    }
  }
  n143 = while {
    shift-right: [w381] -> w4
    shift-left: w1 -> [w384]
    tunnel: w2 -> [w385]
    stop <- w382 stop-if-true
    # "Erzeugerschleife"
    n144 = event shown="[5] \"Test User\": Wertänderung" {
      selector: _ -> [_ _ _ _ _ _]
      dyn-events: _ -> [_ _ _ _ _ _]
      timeout: _ -> [_ _ _ _ _ _]
      tunnel: w385 -> [_ w388 w392 w396 w400 w404]
      tunnel: w384 -> [w386 w390 w394 w398 w402 w406]
      tunnel: [w386 w389 w393 w397 w401 w405] -> w381
      tunnel: ["stop" _ _ _ _ _] -> w383
      event "stop": Value Change {
        n145 = event-data() -> ()  [unwired: 1 in, 1 out]
      }
      event "Test Authentication": Value Change {
        n146 = event-data() -> ()  [unwired: 1 in, 2 out]
        n147 = Enqueue Element(queue=w388, element=LabVIEW.Main.Main_Program_Command."Test Authentication" ("Command"), error in (no error)=w390) -> (error out=w389:errorcluster)  [unwired: 1 in, 2 out]
      }
      event "Test Label": Value Change {
        n148 = event-data() -> ()  [unwired: 1 in, 2 out]
        n149 = Enqueue Element(queue=w392, element=LabVIEW.Main.Main_Program_Command."Test Label" ("Command"), error in (no error)=w394) -> (error out=w393:errorcluster)  [unwired: 1 in, 2 out]
      }
      event "Test Product/Serial Number": Value Change {
        n150 = event-data() -> ()  [unwired: 1 in, 2 out]
        n151 = Enqueue Element(queue=w396, element=LabVIEW.Main.Main_Program_Command."Test Product/Serial Number" ("Command"), error in (no error)=w398) -> (error out=w397:errorcluster)  [unwired: 1 in, 2 out]
      }
      event "Test Vorgang/Fertigmeldung": Value Change {
        n152 = event-data() -> ()  [unwired: 1 in, 2 out]
        n153 = Enqueue Element(queue=w400, element=LabVIEW.Main.Main_Program_Command."Test Vorgang/Fertigmeldung" ("Command"), error in (no error)=w402) -> (error out=w401:errorcluster)  [unwired: 1 in, 2 out]
      }
      event "Test User": Value Change {
        n154 = event-data() -> ()  [unwired: 1 in, 2 out]
        n155 = Enqueue Element(queue=w404, element=LabVIEW.Main.Main_Program_Command."Test User" ("Command"), error in (no error)=w406) -> (error out=w405:errorcluster)  [unwired: 1 in, 2 out]
      }
    }
    n156 = Or(x=w381, y=w383) -> (x .or. y?=w382:bool)
  }
  n157 = Release Queue(queue=w2, error in (no error)=w4) -> ()  [unwired: 1 in, 3 out]
